vi "Test CIF pcap PubSub.vi"() -> ()   [LabVIEW 2021]
uses:
  typedef/CIF Pcap Publisher Configuration.ctl
  typedef/CIF Pcap Subscriber Configuration.ctl
  typedef/CIF Channel Header Publisher.ctl
  typedef/CIF Channel Header.ctl
  typedef/Publisher Info.ctl
  typedef/CIF Pcap Publish Advanced.ctl
  typedef/CIF Pcap Publisher Stats.ctl
  typedef/CIF Pcap Subscriber Stats.ctl
  SubVIs/Get Path.vi
  SubVIs/Convert Error.vi
  SubVIs/Add Error.vi
  Refnum/CIF Publisher to Refnum.vi
  <vilib>/CIF Foundation/CIF Utilities/File/File/File Not Found Error Update.vi
  Refnum/CIF Subscriber to Refnum.vi
  SubVIs/Check data length for publish.vi
  Refnum/CIF Publisher from Refnum.vi
  Refnum/CIF Subscriber from Refnum.vi
  <vilib>/Utility/error.llb/Trim Whitespace.vi
  SubVIs/Add Error Core.vi
  SubVIs/Convert Error Core.vi
  <vilib>/CIF Foundation/CIF Utilities/File/SubVIs/File Not Found Error Core.vi
  Iceoryx.lvlib
panel:
  out "status":string
  out "pass":bool
  out "error out":errorcluster
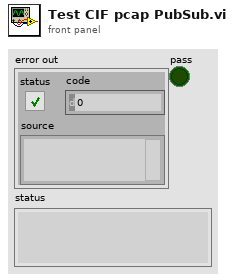
[diagram p1: front panel]
types:
  T1 = typedef "Iceoryx.lvlib/CIF Channel Header.ctl" = cluster{"Length":u64, "T0":i64, "T_Out":i64, "T_Tx":i64, "Ctr":u64, "ClockID":u8}
  T2 = typedef "Iceoryx.lvlib/CIF Channel Header Publisher.ctl" = cluster{"T0":i64, "T_Out":i64, "T_Tx":i64, "ClockID":u8}
  T3 = typedef "Iceoryx.lvlib/CIF Pcap Subscriber Configuration.ctl" = cluster{"Name":string, "Topic":string, "Link Type":u32, "Backpressure":bool}
  T4 = typedef "Iceoryx.lvlib/CIF Pcap Publisher Configuration.ctl" = cluster{"Name":string, "Topic":string, "Link Type":u32, "Descriptor":string, "Max Bytes":u32, "Best Effort Subscribers":u32, "Backpressure Subscribers":u32, "Best Effort Queue Depth":u32, "Backpressure Queue Depth":u32}
  T5 = typedef "Iceoryx.lvlib/Publisher Info.ctl" = cluster{"Type":string, "Element Size":u32, "Max Elements in Array":u32, "Backpressure Queue Depth":u32, "Best Effort Queue Depth":u32}
  T6 = typedef "Iceoryx.lvlib/CIF Pcap Publish Advanced.ctl" = cluster{"Offset":u32, "Length":i32}
  T7 = typedef "Iceoryx.lvlib/CIF Pcap Publisher Stats.ctl" = cluster{"Writes":u64, "TX Timeouts":u64}
  T8 = typedef "Iceoryx.lvlib/CIF Pcap Subscriber Stats.ctl" = cluster{"Reads":u64, "RX Timeouts":u64, "Dropped":u64}
  T9 = typedef "Iceoryx.lvlib/CIF Publisher Refnum.ctl" = cluster{"refnum":u64, "CIF Pub":enum8{"cifpub"}}
  T10 = typedef "Iceoryx.lvlib/CIF Subscriber Refnum.ctl" = cluster{"refnum":u64, "CIF Sub":enum8{"cifsub"}}
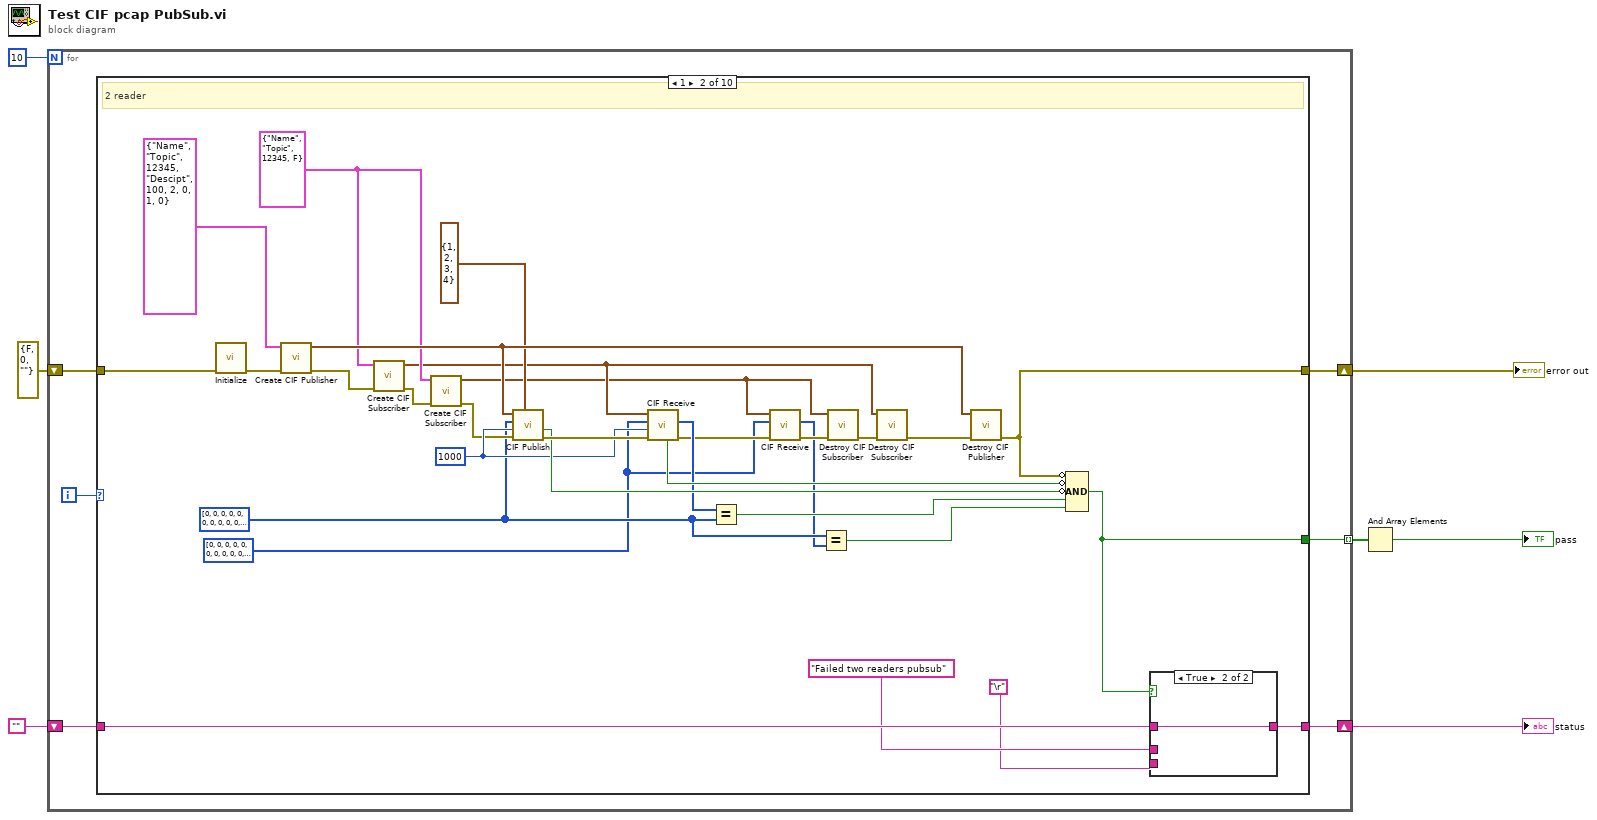
[diagram p0: block diagram]
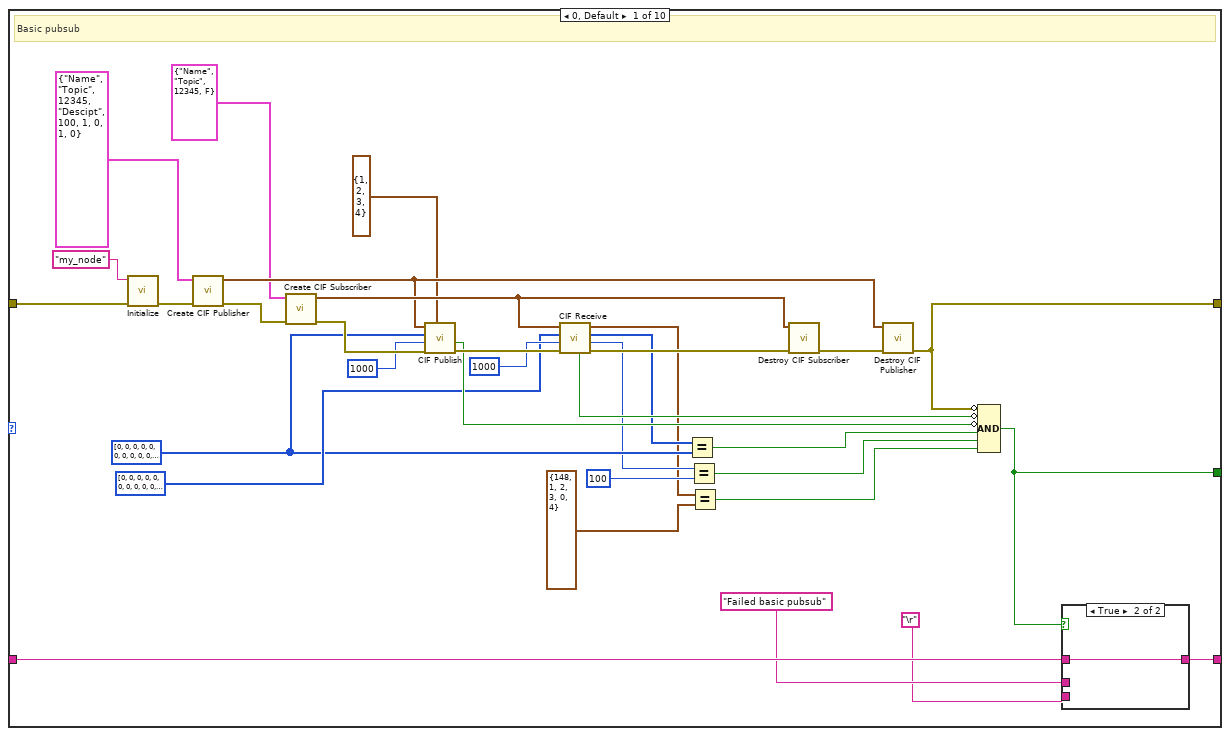
[diagram p2: hidden frame]
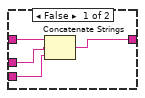
[diagram p3: hidden frame]
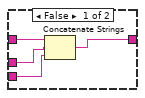
[diagram p4: hidden frame]
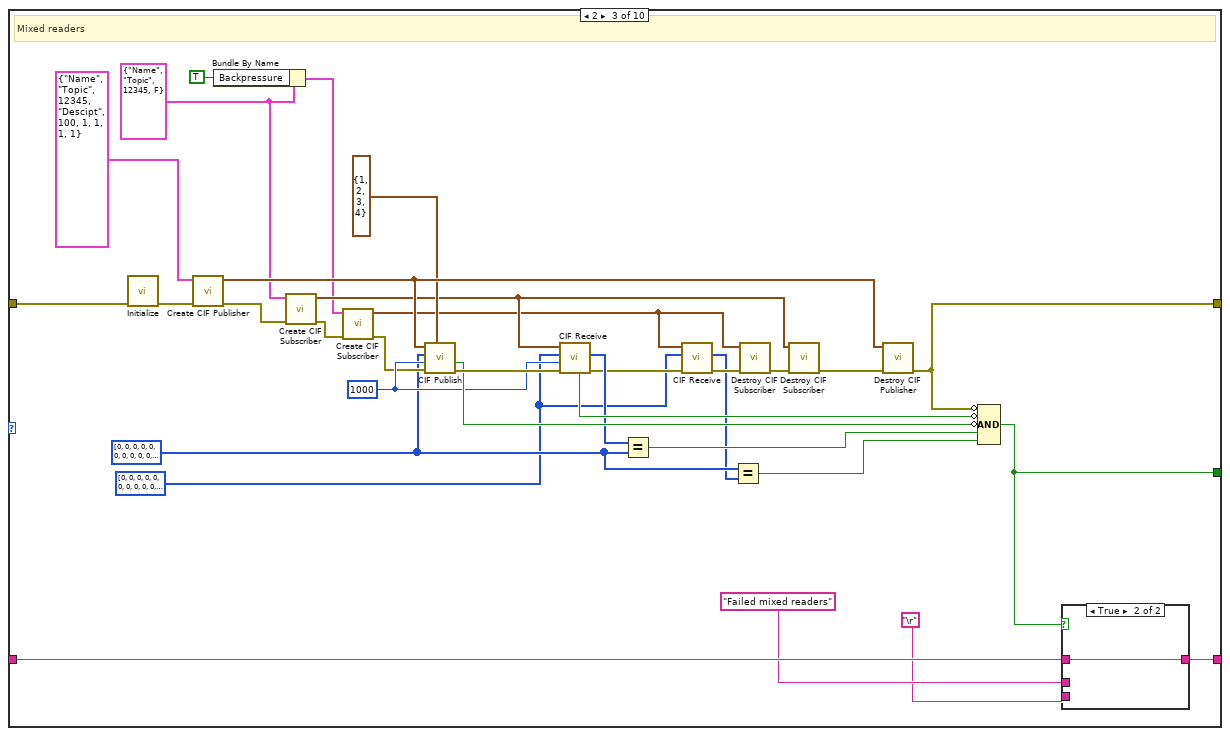
[diagram p5: hidden frame]
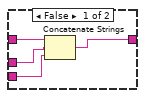
[diagram p6: hidden frame]
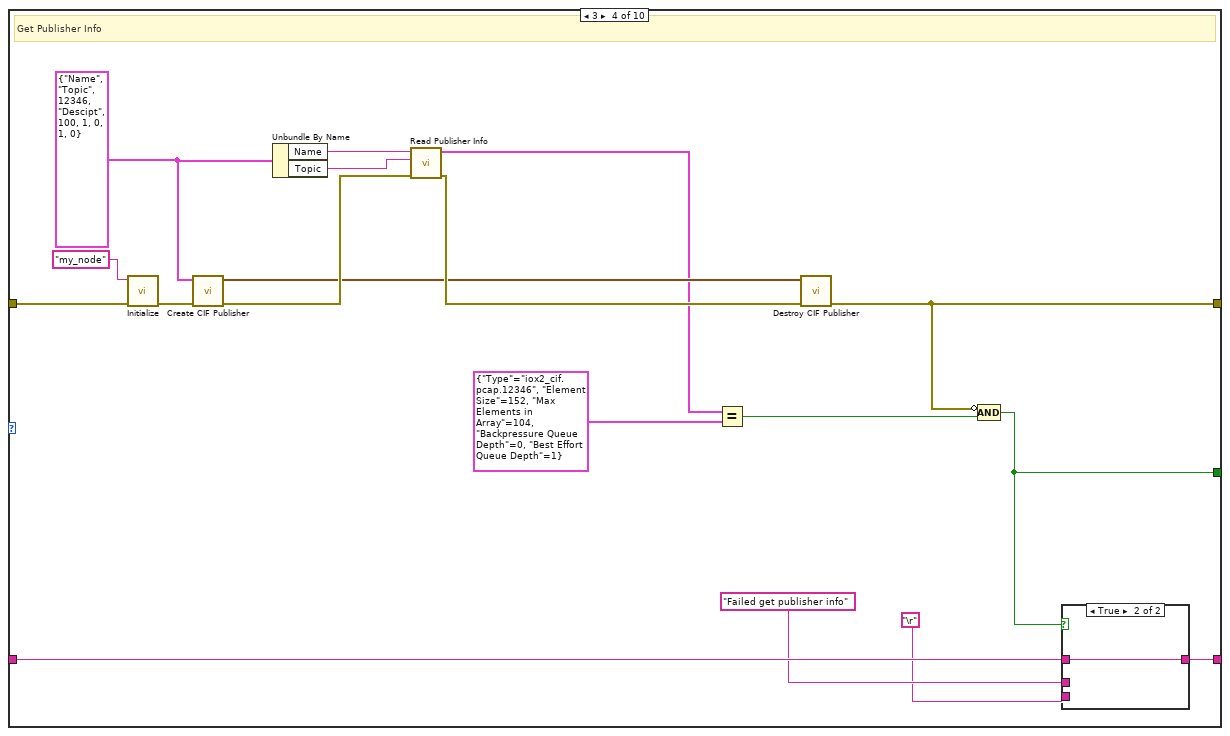
[diagram p7: hidden frame]
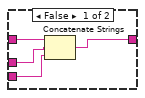
[diagram p8: hidden frame]
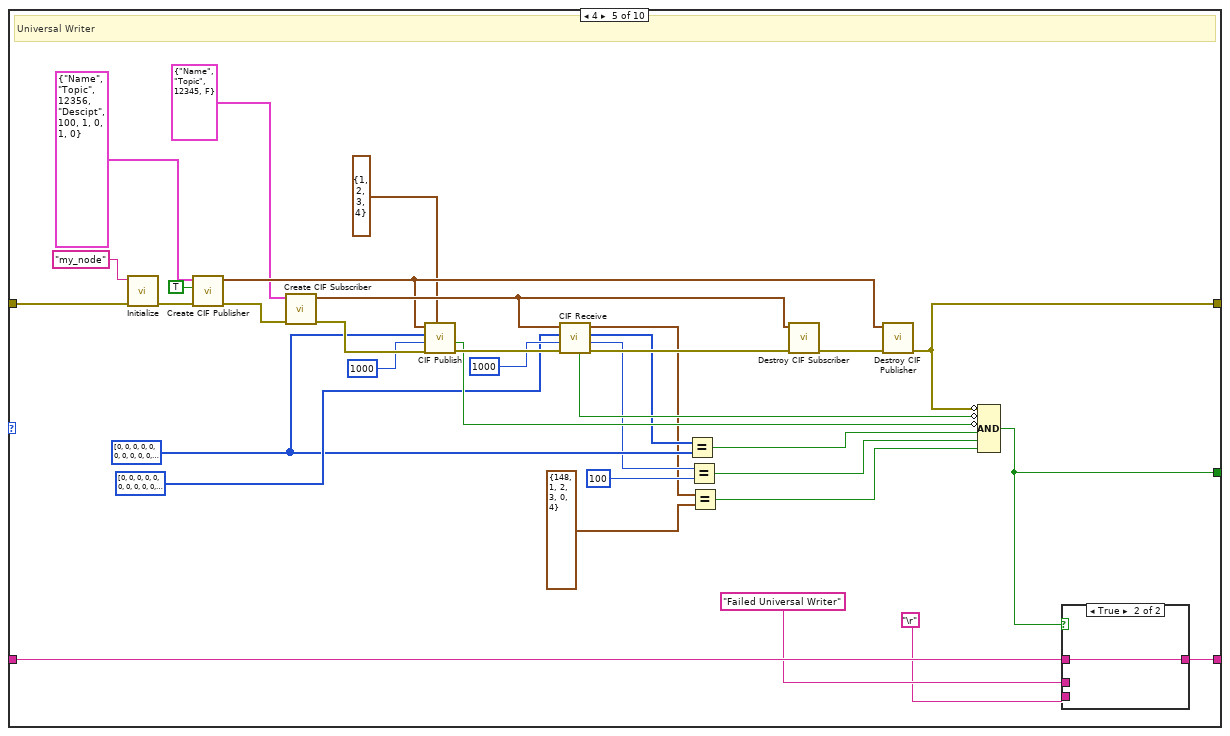
[diagram p9: hidden frame]
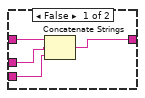
[diagram p10: hidden frame]
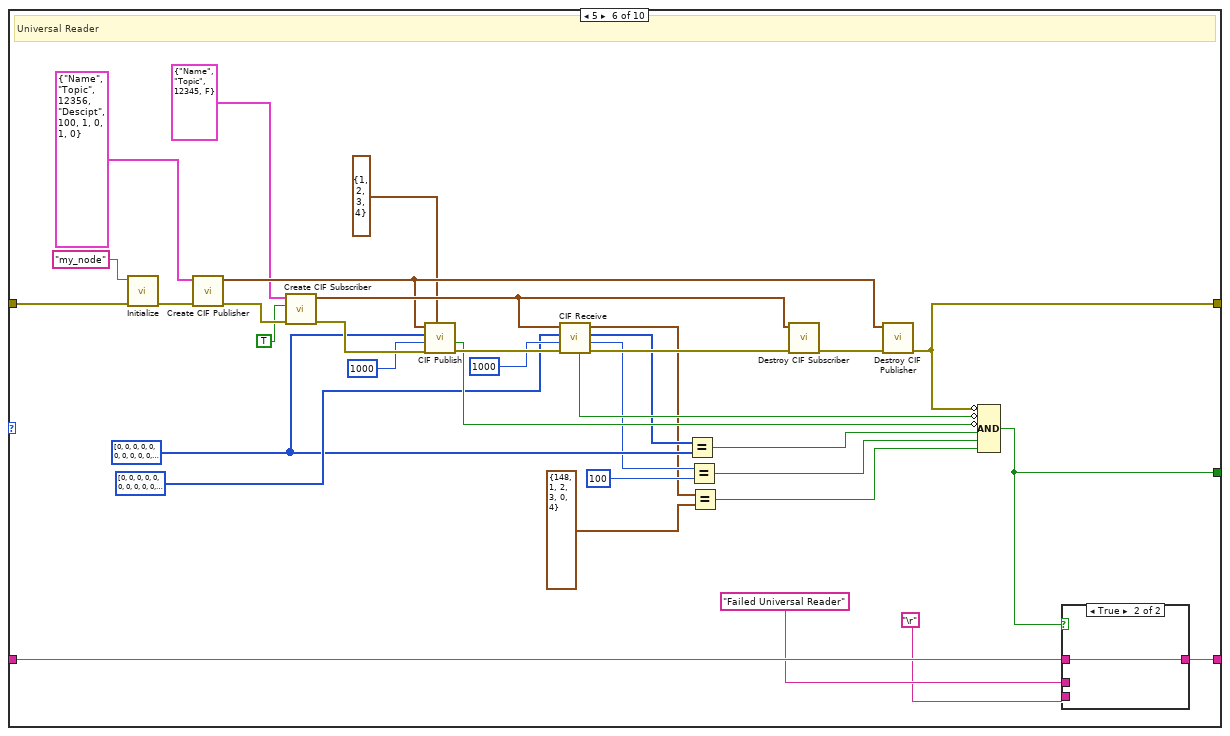
[diagram p11: hidden frame]
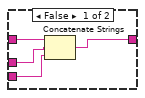
[diagram p12: hidden frame]
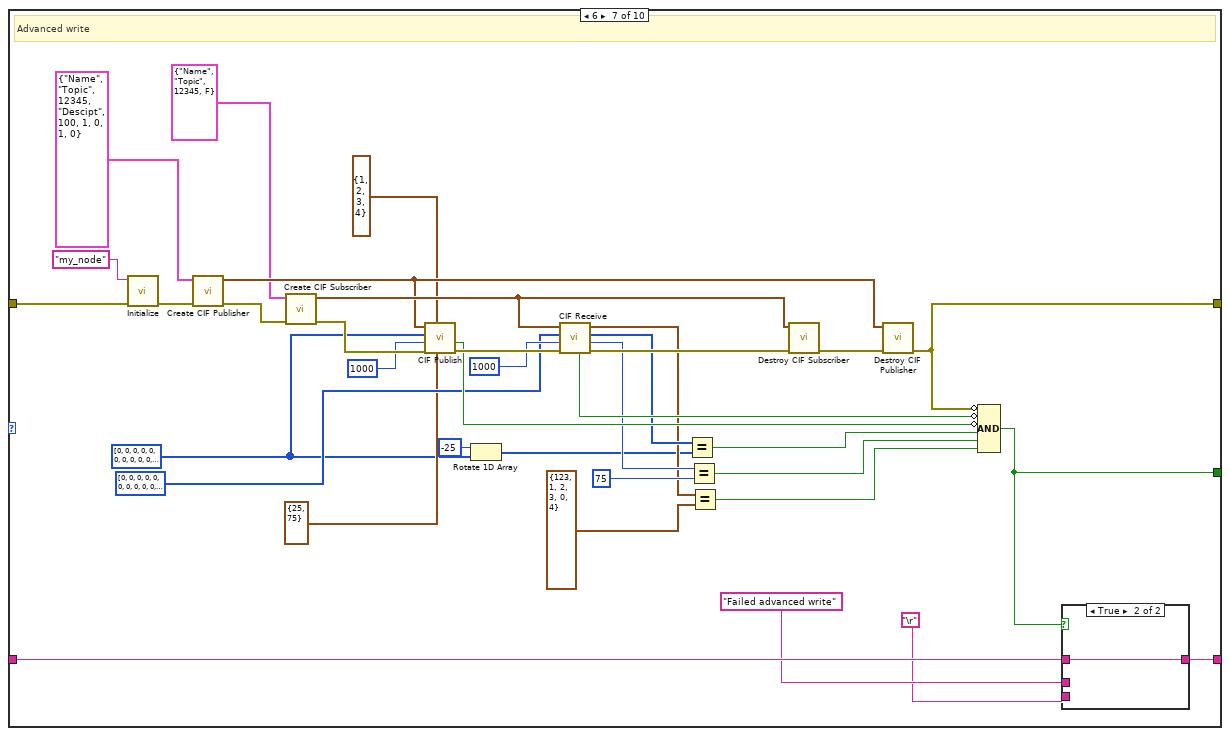
[diagram p13: hidden frame]
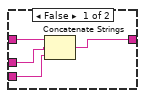
[diagram p14: hidden frame]
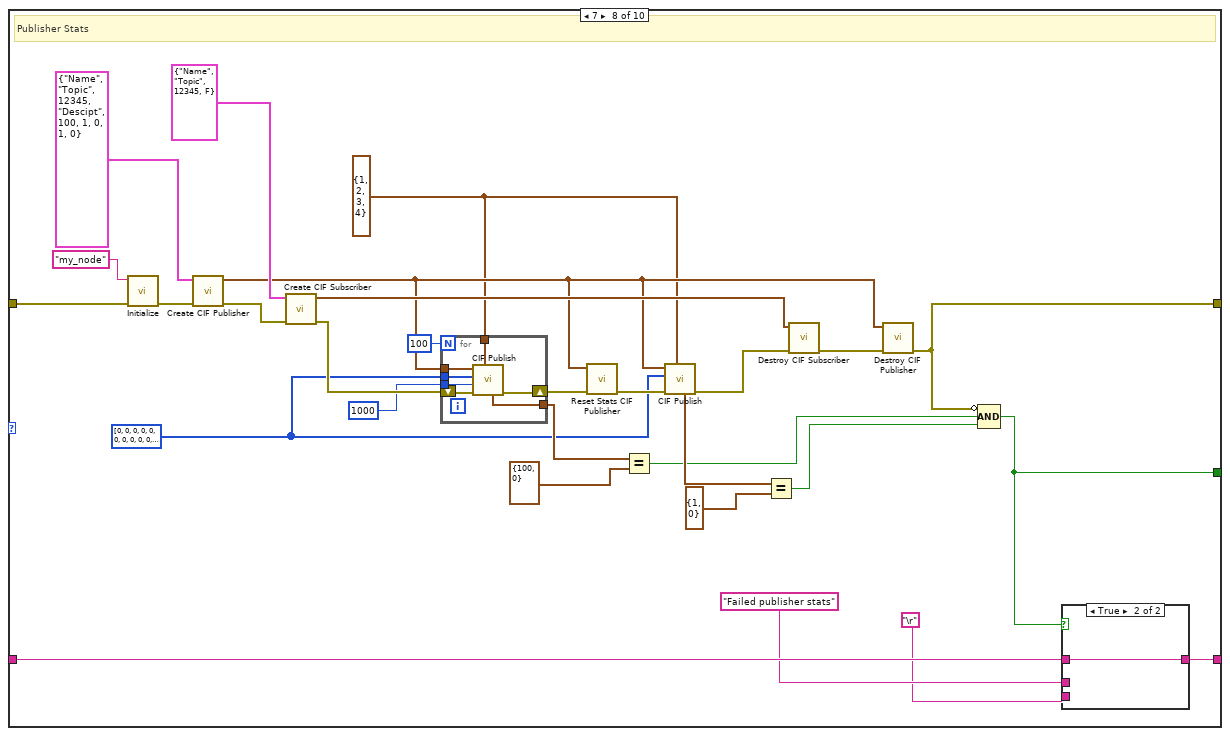
[diagram p15: hidden frame]
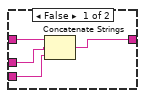
[diagram p16: hidden frame]
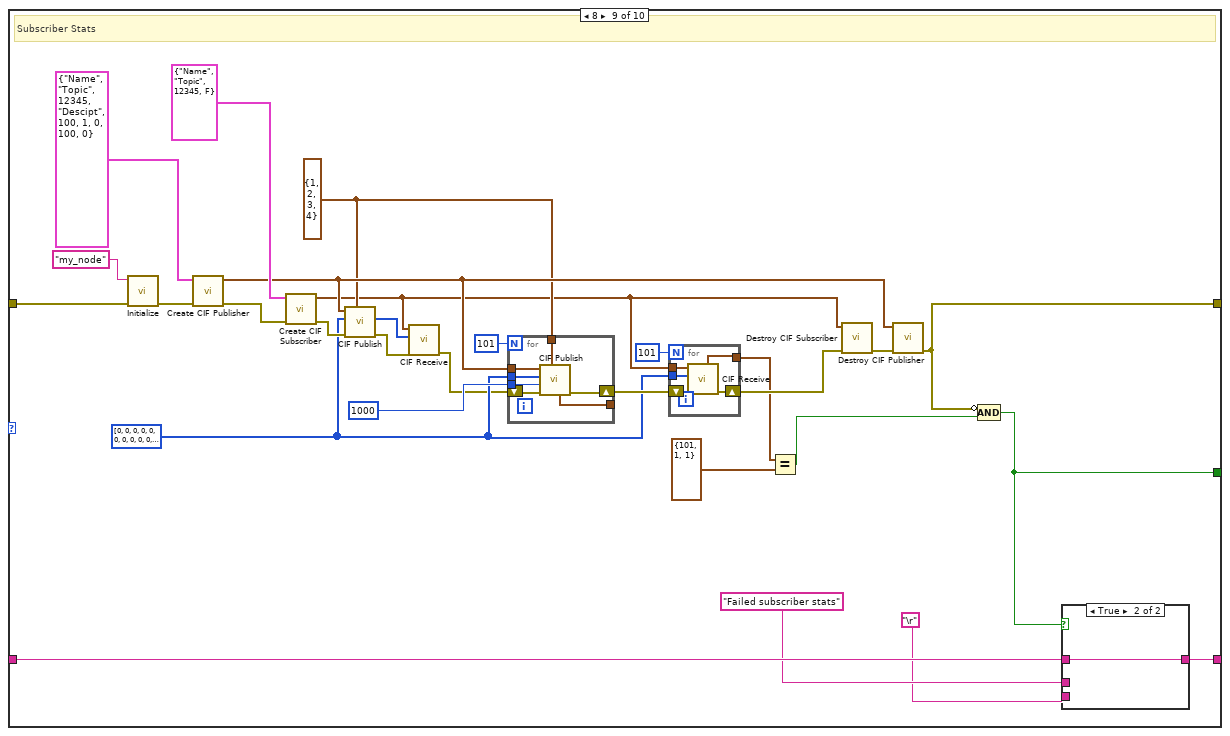
[diagram p17: hidden frame]
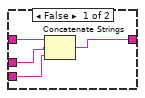
[diagram p18: hidden frame]
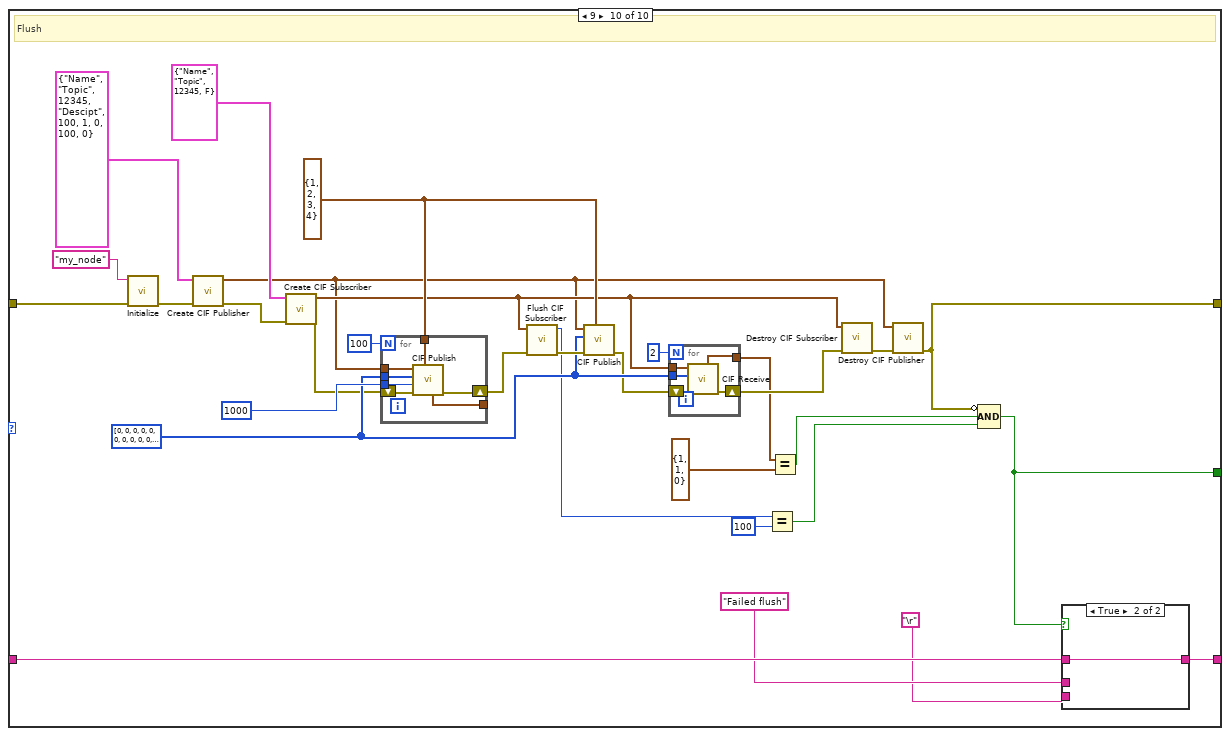
[diagram p19: hidden frame]
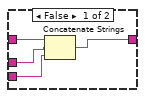
[diagram p20: hidden frame]
diagram:
  n1 = for {
    N: 10 -> [_]
    tunnel: [w13] -> w7 mode=indexing
    shift-right: [w10] -> w3
    shift-left: "" -> [w11]
    shift-right: [w9] -> w1
    shift-left: errorcluster {"status"=FALSE, "code"=0, "source"=""} ("error out") -> [w8]
    i -> [w12]
    n2 = case shown="1" w12 {
      tunnel: [w42 w78 w116 w139 w178 w217 w258 w292 w333 w381] -> w13
      tunnel: w11 -> [w46 w82 w120 w143 w182 w221 w262 w296 w337 w385]
      tunnel: [w45 w81 w119 w142 w181 w220 w261 w295 w336 w384] -> w10
      tunnel: [w31 w71 w109 w129 w167 w206 w247 w284 w327 w375] -> w9
      tunnel: w8 -> [w41 w77 w115 w138 w177 w216 w257 w291 w332 w380]
      frame 0, Default {
        w20 = u8[] [0, 0, 0, 0, 0, 0, 0, 0, 0, 0, 0, 0, 0, 0, 0, 0, 0, 0, 0, 0, 0, 0, 0, 0, 0, 0, 0, 0, 0, 0, 0, 0, 0, 0, 0, 0, 0, 0, 0, 0, 0, 0, 0, 0, 0, 0, 0, 0, 0, 0, 0, 0, 0, 0, 0, 0, 0, 0, 0, 0, 0, 0, 0, 0, 0, 0, 0, 0, 0, 0, 0, 0, 0, 0, 0, 0, 0, 0, 0, 0, 0, 0, 0, 0, 0, 0, 0, 0, 0, 0, 0, 0, 0, 0, 0, 0, 0, 0, 0, 1] ("Data In")
        # "Basic pubsub"
        n3 = call "Initialize.vi"("error in (no error)"=w41, "Node name"="my_node") -> ("error out"=w39:errorcluster)  [unwired: 9 in]
        n4 = call "Create CIF Publisher.vi"("error in (no error)"=w39, "CIF Pcap Publisher Configuration"=T4 {"Name"="Name", "Topic"="Topic", "Link Type"=12345, "Descriptor"="Descipt", "Max Bytes"=100, "Best Effort Subscribers"=1, "Backpressure Subscribers"=0, "Best Effort Queue Depth"=1, "Backpressure Queue Depth"=0}) -> ("error out"=w38:errorcluster, "CIF Publisher Refnum"=w32:T9)  [unwired: 8 in]
        n5 = call "Create CIF Subscriber.vi"("error in (no error)"=w38, "CIF Pcap Subscriber Configuration"=T3 {"Name"="Name", "Topic"="Topic", "Link Type"=12345, "Backpressure"=FALSE}) -> ("error out"=w37:errorcluster, "CIF Subscriber Refnum"=w34:T10)  [unwired: 8 in]
        n6 = call "CIF Publish.vi"("CIF Channel Header Publisher"=T2 {"T0"=1, "T_Out"=2, "T_Tx"=3, "ClockID"=4}, "error in (no error)"=w37, "Timeout ms"=u32 1000 ("Timoeut ms"), "Data In"=w20, "Publisher Reference"=w32) -> ("error out"=w36:errorcluster, "Timeout"=w27:bool)  [unwired: 3 in, 2 out]
        n7 = call "CIF Receive.vi"("error in (no error)"=w36, "Timoeut ms"=u32 1000, "Data In"=u8[] [0, 0, 0, 0, 0, 0, 0, 0, 0, 0, 0, 0, 0, 0, 0, 0, 0, 0, 0, 0, 0, 0, 0, 0, 0, 0, 0, 0, 0, 0, 0, 0, 0, 0, 0, 0, 0, 0, 0, 0, 0, 0, 0, 0, 0, 0, 0, 0, 0, 0, 0, 0, 0, 0, 0, 0, 0, 0, 0, 0, 0, 0, 0, 0, 0, 0, 0, 0, 0, 0, 0, 0, 0, 0, 0, 0, 0, 0, 0, 0, 0, 0, 0, 0, 0, 0, 0, 0, 0, 0, 0, 0, 0, 0, 0, 0, 0, 0, 0, 0], "Subscriber Reference"=w34) -> ("error out"=w35:errorcluster, "Array Length"=w19:u32, "Data Out"=w21:u8[], "CIF Channel Header"=w16:T1, "Timeout"=w26:bool)  [unwired: 2 in, 1 out]
        n8 = Equal?(x=w21, y=w20) -> (x = y?=w28:bool)
        n9 = Equal?(x=w19, y=u32 100) -> (x = y?=w17:bool)
        n10 = Equal?(x=w16, y=T1 {"Length"=148, "T0"=1, "T_Out"=2, "T_Tx"=3, "Ctr"=0, "ClockID"=4} ("CIF Channel Header")) -> (x = y?=w15:bool)
        n11 = call "Destroy CIF Subscriber.vi"("error in (no error)"=w35, "Subscriber Reference"=w34) -> ("error out"=w33:errorcluster)  [unwired: 9 in]
        n12 = call "Destroy CIF Publisher.vi"("error in (no error)"=w33, "Publisher Reference"=w32) -> ("error out"=w31:errorcluster)  [unwired: 9 in]
        n13 = Compound Arithmetic op=AND(invert w31, invert w26, invert w27, w28, w17, w15) -> (w42:bool)
        n14 = case shown="True" w42 {
          tunnel: w46 -> [w50 w51]
          tunnel: [w47 w51] -> w45
          tunnel: "Failed basic pubsub" -> [w49 _]
          tunnel: "\r" -> [w48 _]
          frame False {
            n15 = Concatenate Strings(w50, w49, w48) -> (w47:string)
          }
          frame True {
          }
        }
      }
      frame 1 {
        w52 = u8[] [0, 0, 0, 0, 0, 0, 0, 0, 0, 0, 0, 0, 0, 0, 0, 0, 0, 0, 0, 0, 0, 0, 0, 0, 0, 0, 0, 0, 0, 0, 0, 0, 0, 0, 0, 0, 0, 0, 0, 0, 0, 0, 0, 0, 0, 0, 0, 0, 0, 0, 0, 0, 0, 0, 0, 0, 0, 0, 0, 0, 0, 0, 0, 0, 0, 0, 0, 0, 0, 0, 0, 0, 0, 0, 0, 0, 0, 0, 0, 0, 0, 0, 0, 0, 0, 0, 0, 0, 0, 0, 0, 0, 0, 0, 0, 0, 0, 0, 0, 0] ("Data In")
        w55 = u8[] [0, 0, 0, 0, 0, 0, 0, 0, 0, 0, 0, 0, 0, 0, 0, 0, 0, 0, 0, 0, 0, 0, 0, 0, 0, 0, 0, 0, 0, 0, 0, 0, 0, 0, 0, 0, 0, 0, 0, 0, 0, 0, 0, 0, 0, 0, 0, 0, 0, 0, 0, 0, 0, 0, 0, 0, 0, 0, 0, 0, 0, 0, 0, 0, 0, 0, 0, 0, 0, 0, 0, 0, 0, 0, 0, 0, 0, 0, 0, 0, 0, 0, 0, 0, 0, 0, 0, 0, 0, 0, 0, 0, 0, 0, 0, 0, 0, 0, 0, 1] ("Data In")
        w60 = T3 {"Name"="Name", "Topic"="Topic", "Link Type"=12345, "Backpressure"=FALSE} ("CIF Pcap Subscriber Configuration")
        w63 = u32 1000 ("Timoeut ms")
        # "2 reader"
        n16 = call "Initialize.vi"("error in (no error)"=w77) -> ("error out"=w76:errorcluster)  [unwired: 10 in]
        n17 = call "Create CIF Publisher.vi"("error in (no error)"=w76, "CIF Pcap Publisher Configuration"=T4 {"Name"="Name", "Topic"="Topic", "Link Type"=12345, "Descriptor"="Descipt", "Max Bytes"=100, "Best Effort Subscribers"=2, "Backpressure Subscribers"=0, "Best Effort Queue Depth"=1, "Backpressure Queue Depth"=0}) -> ("error out"=w75:errorcluster, "CIF Publisher Refnum"=w72:T9)  [unwired: 8 in]
        n18 = call "Create CIF Subscriber.vi"("error in (no error)"=w75, "CIF Pcap Subscriber Configuration"=w60) -> ("error out"=w62:errorcluster, "CIF Subscriber Refnum"=w56:T10)  [unwired: 8 in]
        n19 = call "Create CIF Subscriber.vi"("error in (no error)"=w62, "CIF Pcap Subscriber Configuration"=w60) -> ("error out"=w61:errorcluster, "CIF Subscriber Refnum"=w53:T10)  [unwired: 8 in]
        n20 = call "CIF Publish.vi"("CIF Channel Header Publisher"=T2 {"T0"=1, "T_Out"=2, "T_Tx"=3, "ClockID"=4}, "error in (no error)"=w61, "Timeout ms"=w63, "Data In"=w55, "Publisher Reference"=w72) -> ("error out"=w74:errorcluster, "Timeout"=w69:bool)  [unwired: 3 in, 2 out]
        n21 = call "CIF Receive.vi"("error in (no error)"=w74, "Timoeut ms"=w63, "Data In"=w52, "Subscriber Reference"=w56) -> ("error out"=w59:errorcluster, "Data Out"=w65:u8[], "Timeout"=w68:bool)  [unwired: 2 in, 3 out]
        n22 = Equal?(x=w65, y=w55) -> (x = y?=w70:bool)
        n23 = call "CIF Receive.vi"("error in (no error)"=w59, "Data In"=w52, "Subscriber Reference"=w53) -> ("error out"=w58:errorcluster, "Data Out"=w54:u8[])  [unwired: 3 in, 4 out]
        n24 = Equal?(x=w55, y=w54) -> (x = y?=w64:bool)
        n25 = call "Destroy CIF Subscriber.vi"("error in (no error)"=w58, "Subscriber Reference"=w53) -> ("error out"=w57:errorcluster)  [unwired: 9 in]
        n26 = call "Destroy CIF Subscriber.vi"("error in (no error)"=w57, "Subscriber Reference"=w56) -> ("error out"=w73:errorcluster)  [unwired: 9 in]
        n27 = call "Destroy CIF Publisher.vi"("error in (no error)"=w73, "Publisher Reference"=w72) -> ("error out"=w71:errorcluster)  [unwired: 9 in]
        n28 = Compound Arithmetic op=AND(invert w71, invert w68, invert w69, w70, w64) -> (w78:bool)
        n29 = case shown="True" w78 {
          tunnel: w82 -> [w86 w87]
          tunnel: [w83 w87] -> w81
          tunnel: "Failed two readers pubsub" -> [w85 _]
          tunnel: "\r" -> [w84 _]
          frame False {
            n30 = Concatenate Strings(w86, w85, w84) -> (w83:string)
          }
          frame True {
          }
        }
      }
      frame 2 {
        w91 = u8[] [0, 0, 0, 0, 0, 0, 0, 0, 0, 0, 0, 0, 0, 0, 0, 0, 0, 0, 0, 0, 0, 0, 0, 0, 0, 0, 0, 0, 0, 0, 0, 0, 0, 0, 0, 0, 0, 0, 0, 0, 0, 0, 0, 0, 0, 0, 0, 0, 0, 0, 0, 0, 0, 0, 0, 0, 0, 0, 0, 0, 0, 0, 0, 0, 0, 0, 0, 0, 0, 0, 0, 0, 0, 0, 0, 0, 0, 0, 0, 0, 0, 0, 0, 0, 0, 0, 0, 0, 0, 0, 0, 0, 0, 0, 0, 0, 0, 0, 0, 0] ("Data In")
        w94 = u8[] [0, 0, 0, 0, 0, 0, 0, 0, 0, 0, 0, 0, 0, 0, 0, 0, 0, 0, 0, 0, 0, 0, 0, 0, 0, 0, 0, 0, 0, 0, 0, 0, 0, 0, 0, 0, 0, 0, 0, 0, 0, 0, 0, 0, 0, 0, 0, 0, 0, 0, 0, 0, 0, 0, 0, 0, 0, 0, 0, 0, 0, 0, 0, 0, 0, 0, 0, 0, 0, 0, 0, 0, 0, 0, 0, 0, 0, 0, 0, 0, 0, 0, 0, 0, 0, 0, 0, 0, 0, 0, 0, 0, 0, 0, 0, 0, 0, 0, 0, 1] ("Data In")
        w89 = T3 {"Name"="Name", "Topic"="Topic", "Link Type"=12345, "Backpressure"=FALSE} ("CIF Pcap Subscriber Configuration")
        w101 = u32 1000 ("Timoeut ms")
        # "Mixed readers"
        n31 = call "Initialize.vi"("error in (no error)"=w115) -> ("error out"=w114:errorcluster)  [unwired: 10 in]
        n32 = call "Create CIF Publisher.vi"("error in (no error)"=w114, "CIF Pcap Publisher Configuration"=T4 {"Name"="Name", "Topic"="Topic", "Link Type"=12345, "Descriptor"="Descipt", "Max Bytes"=100, "Best Effort Subscribers"=1, "Backpressure Subscribers"=1, "Best Effort Queue Depth"=1, "Backpressure Queue Depth"=1}) -> ("error out"=w113:errorcluster, "CIF Publisher Refnum"=w110:T9)  [unwired: 8 in]
        n33 = Bundle By Name(cluster=w89, "Backpressure"=TRUE) -> (w88:T3)
        n34 = call "Create CIF Subscriber.vi"("error in (no error)"=w113, "CIF Pcap Subscriber Configuration"=w89) -> ("error out"=w100:errorcluster, "CIF Subscriber Refnum"=w95:T10)  [unwired: 8 in]
        n35 = call "Create CIF Subscriber.vi"("error in (no error)"=w100, "CIF Pcap Subscriber Configuration"=w88) -> ("error out"=w99:errorcluster, "CIF Subscriber Refnum"=w92:T10)  [unwired: 8 in]
        n36 = call "CIF Publish.vi"("CIF Channel Header Publisher"=T2 {"T0"=1, "T_Out"=2, "T_Tx"=3, "ClockID"=4}, "error in (no error)"=w99, "Timeout ms"=w101, "Data In"=w94, "Publisher Reference"=w110) -> ("error out"=w112:errorcluster, "Timeout"=w107:bool)  [unwired: 3 in, 2 out]
        n37 = call "CIF Receive.vi"("error in (no error)"=w112, "Timoeut ms"=w101, "Data In"=w91, "Subscriber Reference"=w95) -> ("error out"=w98:errorcluster, "Data Out"=w103:u8[], "Timeout"=w106:bool)  [unwired: 2 in, 3 out]
        n38 = Equal?(x=w103, y=w94) -> (x = y?=w108:bool)
        n39 = call "CIF Receive.vi"("error in (no error)"=w98, "Data In"=w91, "Subscriber Reference"=w92) -> ("error out"=w97:errorcluster, "Data Out"=w93:u8[])  [unwired: 3 in, 4 out]
        n40 = Equal?(x=w94, y=w93) -> (x = y?=w102:bool)
        n41 = call "Destroy CIF Subscriber.vi"("error in (no error)"=w97, "Subscriber Reference"=w92) -> ("error out"=w96:errorcluster)  [unwired: 9 in]
        n42 = call "Destroy CIF Subscriber.vi"("error in (no error)"=w96, "Subscriber Reference"=w95) -> ("error out"=w111:errorcluster)  [unwired: 9 in]
        n43 = call "Destroy CIF Publisher.vi"("error in (no error)"=w111, "Publisher Reference"=w110) -> ("error out"=w109:errorcluster)  [unwired: 9 in]
        n44 = Compound Arithmetic op=AND(invert w109, invert w106, invert w107, w108, w102) -> (w116:bool)
        n45 = case shown="True" w116 {
          tunnel: w120 -> [w124 w125]
          tunnel: [w121 w125] -> w119
          tunnel: "Failed mixed readers" -> [w123 _]
          tunnel: "\r" -> [w122 _]
          frame False {
            n46 = Concatenate Strings(w124, w123, w122) -> (w121:string)
          }
          frame True {
          }
        }
      }
      frame 3 {
        w132 = T4 {"Name"="Name", "Topic"="Topic", "Link Type"=12346, "Descriptor"="Descipt", "Max Bytes"=100, "Best Effort Subscribers"=1, "Backpressure Subscribers"=0, "Best Effort Queue Depth"=1, "Backpressure Queue Depth"=0} ("CIF Pcap Publisher Configuration")
        # "Get Publisher Info"
        n47 = call "Initialize.vi"("error in (no error)"=w138, "Node name"="my_node") -> ("error out"=w136:errorcluster)  [unwired: 9 in]
        n48 = call "Create CIF Publisher.vi"("error in (no error)"=w136, "CIF Pcap Publisher Configuration"=w132) -> ("error out"=w131:errorcluster, "CIF Publisher Refnum"=w128:T9)  [unwired: 8 in]
        n49 = Unbundle By Name(w132) -> ("Name"=w134:string, "Topic"=w133:string)
        n50 = call "Read Publisher Info.vi"("error in (no error)"=w131, "Topic"=w133, "Name"=w134) -> ("error out"=w130:errorcluster, "Publisher Info"=w127:T5)  [unwired: 7 in]
        n51 = Equal?(x=w127, y=T5 {"Type"="iox2_cif.pcap.12346", "Element Size"=152, "Max Elements in Array"=104, "Backpressure Queue Depth"=0, "Best Effort Queue Depth"=1} ("Publisher Info")) -> (x = y?=w135:bool)
        n52 = call "Destroy CIF Publisher.vi"("error in (no error)"=w130, "Publisher Reference"=w128) -> ("error out"=w129:errorcluster)  [unwired: 9 in]
        n53 = Compound Arithmetic op=AND(invert w129, w135) -> (w139:bool)
        n54 = case shown="True" w139 {
          tunnel: w143 -> [w147 w148]
          tunnel: [w144 w148] -> w142
          tunnel: "Failed get publisher info" -> [w146 _]
          tunnel: "\r" -> [w145 _]
          frame False {
            n55 = Concatenate Strings(w147, w146, w145) -> (w144:string)
          }
          frame True {
          }
        }
      }
      frame 4 {
        w156 = u8[] [0, 0, 0, 0, 0, 0, 0, 0, 0, 0, 0, 0, 0, 0, 0, 0, 0, 0, 0, 0, 0, 0, 0, 0, 0, 0, 0, 0, 0, 0, 0, 0, 0, 0, 0, 0, 0, 0, 0, 0, 0, 0, 0, 0, 0, 0, 0, 0, 0, 0, 0, 0, 0, 0, 0, 0, 0, 0, 0, 0, 0, 0, 0, 0, 0, 0, 0, 0, 0, 0, 0, 0, 0, 0, 0, 0, 0, 0, 0, 0, 0, 0, 0, 0, 0, 0, 0, 0, 0, 0, 0, 0, 0, 0, 0, 0, 0, 0, 0, 1] ("Data In")
        # "Universal Writer"
        n56 = call "Initialize.vi"("error in (no error)"=w177, "Node name"="my_node") -> ("error out"=w175:errorcluster)  [unwired: 9 in]
        n57 = call "Create CIF Publisher.vi"("error in (no error)"=w175, "Universal"=TRUE, "CIF Pcap Publisher Configuration"=T4 {"Name"="Name", "Topic"="Topic", "Link Type"=12356, "Descriptor"="Descipt", "Max Bytes"=100, "Best Effort Subscribers"=1, "Backpressure Subscribers"=0, "Best Effort Queue Depth"=1, "Backpressure Queue Depth"=0}) -> ("error out"=w174:errorcluster, "CIF Publisher Refnum"=w168:T9)  [unwired: 7 in]
        n58 = call "Create CIF Subscriber.vi"("error in (no error)"=w174, "CIF Pcap Subscriber Configuration"=T3 {"Name"="Name", "Topic"="Topic", "Link Type"=12345, "Backpressure"=FALSE}) -> ("error out"=w173:errorcluster, "CIF Subscriber Refnum"=w170:T10)  [unwired: 8 in]
        n59 = call "CIF Publish.vi"("CIF Channel Header Publisher"=T2 {"T0"=1, "T_Out"=2, "T_Tx"=3, "ClockID"=4}, "error in (no error)"=w173, "Timeout ms"=u32 1000 ("Timoeut ms"), "Data In"=w156, "Publisher Reference"=w168) -> ("error out"=w172:errorcluster, "Timeout"=w163:bool)  [unwired: 3 in, 2 out]
        n60 = call "CIF Receive.vi"("error in (no error)"=w172, "Timoeut ms"=u32 1000, "Data In"=u8[] [0, 0, 0, 0, 0, 0, 0, 0, 0, 0, 0, 0, 0, 0, 0, 0, 0, 0, 0, 0, 0, 0, 0, 0, 0, 0, 0, 0, 0, 0, 0, 0, 0, 0, 0, 0, 0, 0, 0, 0, 0, 0, 0, 0, 0, 0, 0, 0, 0, 0, 0, 0, 0, 0, 0, 0, 0, 0, 0, 0, 0, 0, 0, 0, 0, 0, 0, 0, 0, 0, 0, 0, 0, 0, 0, 0, 0, 0, 0, 0, 0, 0, 0, 0, 0, 0, 0, 0, 0, 0, 0, 0, 0, 0, 0, 0, 0, 0, 0, 0], "Subscriber Reference"=w170) -> ("error out"=w171:errorcluster, "Array Length"=w155:u32, "Data Out"=w157:u8[], "CIF Channel Header"=w152:T1, "Timeout"=w162:bool)  [unwired: 2 in, 1 out]
        n61 = Equal?(x=w157, y=w156) -> (x = y?=w164:bool)
        n62 = Equal?(x=w155, y=u32 100) -> (x = y?=w153:bool)
        n63 = Equal?(x=w152, y=T1 {"Length"=148, "T0"=1, "T_Out"=2, "T_Tx"=3, "Ctr"=0, "ClockID"=4} ("CIF Channel Header")) -> (x = y?=w151:bool)
        n64 = call "Destroy CIF Subscriber.vi"("error in (no error)"=w171, "Subscriber Reference"=w170) -> ("error out"=w169:errorcluster)  [unwired: 9 in]
        n65 = call "Destroy CIF Publisher.vi"("error in (no error)"=w169, "Publisher Reference"=w168) -> ("error out"=w167:errorcluster)  [unwired: 9 in]
        n66 = Compound Arithmetic op=AND(invert w167, invert w162, invert w163, w164, w153, w151) -> (w178:bool)
        n67 = case shown="True" w178 {
          tunnel: w182 -> [w186 w187]
          tunnel: [w183 w187] -> w181
          tunnel: "Failed Universal Writer" -> [w185 _]
          tunnel: "\r" -> [w184 _]
          frame False {
            n68 = Concatenate Strings(w186, w185, w184) -> (w183:string)
          }
          frame True {
          }
        }
      }
      frame 5 {
        w195 = u8[] [0, 0, 0, 0, 0, 0, 0, 0, 0, 0, 0, 0, 0, 0, 0, 0, 0, 0, 0, 0, 0, 0, 0, 0, 0, 0, 0, 0, 0, 0, 0, 0, 0, 0, 0, 0, 0, 0, 0, 0, 0, 0, 0, 0, 0, 0, 0, 0, 0, 0, 0, 0, 0, 0, 0, 0, 0, 0, 0, 0, 0, 0, 0, 0, 0, 0, 0, 0, 0, 0, 0, 0, 0, 0, 0, 0, 0, 0, 0, 0, 0, 0, 0, 0, 0, 0, 0, 0, 0, 0, 0, 0, 0, 0, 0, 0, 0, 0, 0, 1] ("Data In")
        # "Universal Reader"
        n69 = call "Initialize.vi"("error in (no error)"=w216, "Node name"="my_node") -> ("error out"=w214:errorcluster)  [unwired: 9 in]
        n70 = call "Create CIF Publisher.vi"("error in (no error)"=w214, "CIF Pcap Publisher Configuration"=T4 {"Name"="Name", "Topic"="Topic", "Link Type"=12356, "Descriptor"="Descipt", "Max Bytes"=100, "Best Effort Subscribers"=1, "Backpressure Subscribers"=0, "Best Effort Queue Depth"=1, "Backpressure Queue Depth"=0}) -> ("error out"=w213:errorcluster, "CIF Publisher Refnum"=w207:T9)  [unwired: 8 in]
        n71 = call "Create CIF Subscriber.vi"("error in (no error)"=w213, "Universal"=TRUE, "CIF Pcap Subscriber Configuration"=T3 {"Name"="Name", "Topic"="Topic", "Link Type"=12345, "Backpressure"=FALSE}) -> ("error out"=w212:errorcluster, "CIF Subscriber Refnum"=w209:T10)  [unwired: 7 in]
        n72 = call "CIF Publish.vi"("CIF Channel Header Publisher"=T2 {"T0"=1, "T_Out"=2, "T_Tx"=3, "ClockID"=4}, "error in (no error)"=w212, "Timeout ms"=u32 1000 ("Timoeut ms"), "Data In"=w195, "Publisher Reference"=w207) -> ("error out"=w211:errorcluster, "Timeout"=w202:bool)  [unwired: 3 in, 2 out]
        n73 = call "CIF Receive.vi"("error in (no error)"=w211, "Timoeut ms"=u32 1000, "Data In"=u8[] [0, 0, 0, 0, 0, 0, 0, 0, 0, 0, 0, 0, 0, 0, 0, 0, 0, 0, 0, 0, 0, 0, 0, 0, 0, 0, 0, 0, 0, 0, 0, 0, 0, 0, 0, 0, 0, 0, 0, 0, 0, 0, 0, 0, 0, 0, 0, 0, 0, 0, 0, 0, 0, 0, 0, 0, 0, 0, 0, 0, 0, 0, 0, 0, 0, 0, 0, 0, 0, 0, 0, 0, 0, 0, 0, 0, 0, 0, 0, 0, 0, 0, 0, 0, 0, 0, 0, 0, 0, 0, 0, 0, 0, 0, 0, 0, 0, 0, 0, 0], "Subscriber Reference"=w209) -> ("error out"=w210:errorcluster, "Array Length"=w194:u32, "Data Out"=w196:u8[], "CIF Channel Header"=w191:T1, "Timeout"=w201:bool)  [unwired: 2 in, 1 out]
        n74 = Equal?(x=w196, y=w195) -> (x = y?=w203:bool)
        n75 = Equal?(x=w194, y=u32 100) -> (x = y?=w192:bool)
        n76 = Equal?(x=w191, y=T1 {"Length"=148, "T0"=1, "T_Out"=2, "T_Tx"=3, "Ctr"=0, "ClockID"=4} ("CIF Channel Header")) -> (x = y?=w190:bool)
        n77 = call "Destroy CIF Subscriber.vi"("error in (no error)"=w210, "Subscriber Reference"=w209) -> ("error out"=w208:errorcluster)  [unwired: 9 in]
        n78 = call "Destroy CIF Publisher.vi"("error in (no error)"=w208, "Publisher Reference"=w207) -> ("error out"=w206:errorcluster)  [unwired: 9 in]
        n79 = Compound Arithmetic op=AND(invert w206, invert w201, invert w202, w203, w192, w190) -> (w217:bool)
        n80 = case shown="True" w217 {
          tunnel: w221 -> [w225 w226]
          tunnel: [w222 w226] -> w220
          tunnel: "Failed Universal Reader" -> [w224 _]
          tunnel: "\r" -> [w223 _]
          frame False {
            n81 = Concatenate Strings(w225, w224, w223) -> (w222:string)
          }
          frame True {
          }
        }
      }
      frame 6 {
        w229 = u8[] [0, 0, 0, 0, 0, 0, 0, 0, 0, 0, 0, 0, 0, 0, 0, 0, 0, 0, 0, 0, 0, 0, 0, 0, 0, 0, 0, 0, 0, 0, 0, 0, 0, 0, 0, 0, 0, 0, 0, 0, 0, 0, 0, 0, 0, 0, 0, 0, 0, 0, 0, 0, 0, 0, 0, 0, 0, 0, 0, 0, 0, 0, 0, 0, 0, 0, 0, 0, 0, 0, 0, 0, 0, 0, 0, 0, 0, 0, 0, 0, 0, 0, 0, 0, 0, 0, 0, 0, 0, 0, 0, 0, 0, 0, 0, 0, 0, 0, 0, 1] ("Data In")
        # "Advanced write"
        n82 = call "Initialize.vi"("error in (no error)"=w257, "Node name"="my_node") -> ("error out"=w255:errorcluster)  [unwired: 9 in]
        n83 = call "Create CIF Publisher.vi"("error in (no error)"=w255, "CIF Pcap Publisher Configuration"=T4 {"Name"="Name", "Topic"="Topic", "Link Type"=12345, "Descriptor"="Descipt", "Max Bytes"=100, "Best Effort Subscribers"=1, "Backpressure Subscribers"=0, "Best Effort Queue Depth"=1, "Backpressure Queue Depth"=0}) -> ("error out"=w254:errorcluster, "CIF Publisher Refnum"=w248:T9)  [unwired: 8 in]
        n84 = call "Create CIF Subscriber.vi"("error in (no error)"=w254, "CIF Pcap Subscriber Configuration"=T3 {"Name"="Name", "Topic"="Topic", "Link Type"=12345, "Backpressure"=FALSE}) -> ("error out"=w253:errorcluster, "CIF Subscriber Refnum"=w250:T10)  [unwired: 8 in]
        n85 = call "CIF Publish.vi"("CIF Publish Advanced"=T6 {"Offset"=25, "Length"=75}, "CIF Channel Header Publisher"=T2 {"T0"=1, "T_Out"=2, "T_Tx"=3, "ClockID"=4}, "error in (no error)"=w253, "Timeout ms"=u32 1000 ("Timoeut ms"), "Data In"=w229, "Publisher Reference"=w248) -> ("error out"=w252:errorcluster, "Timeout"=w243:bool)  [unwired: 2 in, 2 out]
        n86 = Rotate 1D Array(1:w229, 2:-25 ("n")) -> (0:w227:u8[])
        n87 = call "CIF Receive.vi"("error in (no error)"=w252, "Timoeut ms"=u32 1000, "Data In"=u8[] [0, 0, 0, 0, 0, 0, 0, 0, 0, 0, 0, 0, 0, 0, 0, 0, 0, 0, 0, 0, 0, 0, 0, 0, 0, 0, 0, 0, 0, 0, 0, 0, 0, 0, 0, 0, 0, 0, 0, 0, 0, 0, 0, 0, 0, 0, 0, 0, 0, 0, 0, 0, 0, 0, 0, 0, 0, 0, 0, 0, 0, 0, 0, 0, 0, 0, 0, 0, 0, 0, 0, 0, 0, 0, 0, 0, 0, 0, 0, 0, 0, 0, 0, 0, 0, 0, 0, 0, 0, 0, 0, 0, 0, 0, 0, 0, 0, 0, 0, 0], "Subscriber Reference"=w250) -> ("error out"=w251:errorcluster, "Array Length"=w236:u32, "Data Out"=w237:u8[], "CIF Channel Header"=w233:T1, "Timeout"=w242:bool)  [unwired: 2 in, 1 out]
        n88 = Equal?(x=w237, y=w227) -> (x = y?=w244:bool)
        n89 = Equal?(x=w236, y=u32 75) -> (x = y?=w234:bool)
        n90 = Equal?(x=w233, y=T1 {"Length"=123, "T0"=1, "T_Out"=2, "T_Tx"=3, "Ctr"=0, "ClockID"=4} ("CIF Channel Header")) -> (x = y?=w232:bool)
        n91 = call "Destroy CIF Subscriber.vi"("error in (no error)"=w251, "Subscriber Reference"=w250) -> ("error out"=w249:errorcluster)  [unwired: 9 in]
        n92 = call "Destroy CIF Publisher.vi"("error in (no error)"=w249, "Publisher Reference"=w248) -> ("error out"=w247:errorcluster)  [unwired: 9 in]
        n93 = Compound Arithmetic op=AND(invert w247, invert w242, invert w243, w244, w234, w232) -> (w258:bool)
        n94 = case shown="True" w258 {
          tunnel: w262 -> [w266 w267]
          tunnel: [w263 w267] -> w261
          tunnel: "Failed advanced write" -> [w265 _]
          tunnel: "\r" -> [w264 _]
          frame False {
            n95 = Concatenate Strings(w266, w265, w264) -> (w263:string)
          }
          frame True {
          }
        }
      }
      frame 7 {
        w273 = T2 {"T0"=1, "T_Out"=2, "T_Tx"=3, "ClockID"=4} ("CIF Channel Header Publisher")
        w274 = u8[] [0, 0, 0, 0, 0, 0, 0, 0, 0, 0, 0, 0, 0, 0, 0, 0, 0, 0, 0, 0, 0, 0, 0, 0, 0, 0, 0, 0, 0, 0, 0, 0, 0, 0, 0, 0, 0, 0, 0, 0, 0, 0, 0, 0, 0, 0, 0, 0, 0, 0, 0, 0, 0, 0, 0, 0, 0, 0, 0, 0, 0, 0, 0, 0, 0, 0, 0, 0, 0, 0, 0, 0, 0, 0, 0, 0, 0, 0, 0, 0, 0, 0, 0, 0, 0, 0, 0, 0, 0, 0, 0, 0, 0, 0, 0, 0, 0, 0, 0, 1] ("Data In")
        # "Publisher Stats"
        n96 = call "Initialize.vi"("error in (no error)"=w291, "Node name"="my_node") -> ("error out"=w289:errorcluster)  [unwired: 9 in]
        n97 = call "Create CIF Publisher.vi"("error in (no error)"=w289, "CIF Pcap Publisher Configuration"=T4 {"Name"="Name", "Topic"="Topic", "Link Type"=12345, "Descriptor"="Descipt", "Max Bytes"=100, "Best Effort Subscribers"=1, "Backpressure Subscribers"=0, "Best Effort Queue Depth"=1, "Backpressure Queue Depth"=0}) -> ("error out"=w288:errorcluster, "CIF Publisher Refnum"=w275:T9)  [unwired: 8 in]
        n98 = call "Create CIF Subscriber.vi"("error in (no error)"=w288, "CIF Pcap Subscriber Configuration"=T3 {"Name"="Name", "Topic"="Topic", "Link Type"=12345, "Backpressure"=FALSE}) -> ("error out"=w287:errorcluster, "CIF Subscriber Refnum"=w286:T10)  [unwired: 8 in]
        n99 = for {
          N: 100 -> [_]
          tunnel: w275 -> [w302]
          tunnel: u32 1000 ("Timoeut ms") -> [w301]
          tunnel: w273 -> [w300]
          tunnel: w274 -> [w299]
          tunnel: [w298] -> w278
          shift-right: [w297] -> w277
          shift-left: w287 -> [w303]
          n100 = call "CIF Publish.vi"("CIF Channel Header Publisher"=w300, "error in (no error)"=w303, "Timeout ms"=w301, "Data In"=w299, "Publisher Reference"=w302) -> ("error out"=w297:errorcluster, "CIF Publisher Stats"=w298:T7)  [unwired: 3 in, 2 out]
        }
        n101 = call "Reset Stats CIF Publisher.vi"("error in (no error)"=w277, "Publisher Reference"=w275) -> ("error out"=w276:errorcluster)  [unwired: 9 in]
        n102 = Equal?(x=w278, y=T7 {"Writes"=100, "TX Timeouts"=0} ("CIF Publisher Stats")) -> (x = y?=w269:bool)
        n103 = call "CIF Publish.vi"("CIF Channel Header Publisher"=w273, "error in (no error)"=w276, "Data In"=w274, "Publisher Reference"=w275) -> ("error out"=w270:errorcluster, "CIF Publisher Stats"=w272:T7)  [unwired: 4 in, 2 out]
        n104 = Equal?(x=w272, y=T7 {"Writes"=1, "TX Timeouts"=0} ("CIF Publisher Stats")) -> (x = y?=w268:bool)
        n105 = call "Destroy CIF Subscriber.vi"("error in (no error)"=w270, "Subscriber Reference"=w286) -> ("error out"=w285:errorcluster)  [unwired: 9 in]
        n106 = call "Destroy CIF Publisher.vi"("error in (no error)"=w285, "Publisher Reference"=w275) -> ("error out"=w284:errorcluster)  [unwired: 9 in]
        n107 = Compound Arithmetic op=AND(invert w284, w269, w268) -> (w292:bool)
        n108 = case shown="True" w292 {
          tunnel: w296 -> [w307 w308]
          tunnel: [w304 w308] -> w295
          tunnel: "Failed publisher stats" -> [w306 _]
          tunnel: "\r" -> [w305 _]
          frame False {
            n109 = Concatenate Strings(w307, w306, w305) -> (w304:string)
          }
          frame True {
          }
        }
      }
      frame 8 {
        w314 = T2 {"T0"=1, "T_Out"=2, "T_Tx"=3, "ClockID"=4} ("CIF Channel Header Publisher")
        w313 = u8[] [0, 0, 0, 0, 0, 0, 0, 0, 0, 0, 0, 0, 0, 0, 0, 0, 0, 0, 0, 0, 0, 0, 0, 0, 0, 0, 0, 0, 0, 0, 0, 0, 0, 0, 0, 0, 0, 0, 0, 0, 0, 0, 0, 0, 0, 0, 0, 0, 0, 0, 0, 0, 0, 0, 0, 0, 0, 0, 0, 0, 0, 0, 0, 0, 0, 0, 0, 0, 0, 0, 0, 0, 0, 0, 0, 0, 0, 0, 0, 0, 0, 0, 0, 0, 0, 0, 0, 0, 0, 0, 0, 0, 0, 0, 0, 0, 0, 0, 0, 1] ("Data In")
        # "Subscriber Stats"
        n110 = call "Initialize.vi"("error in (no error)"=w332, "Node name"="my_node") -> ("error out"=w330:errorcluster)  [unwired: 9 in]
        n111 = call "Create CIF Publisher.vi"("error in (no error)"=w330, "CIF Pcap Publisher Configuration"=T4 {"Name"="Name", "Topic"="Topic", "Link Type"=12345, "Descriptor"="Descipt", "Max Bytes"=100, "Best Effort Subscribers"=1, "Backpressure Subscribers"=0, "Best Effort Queue Depth"=100, "Backpressure Queue Depth"=0}) -> ("error out"=w329:errorcluster, "CIF Publisher Refnum"=w316:T9)  [unwired: 8 in]
        n112 = call "Create CIF Subscriber.vi"("error in (no error)"=w329, "CIF Pcap Subscriber Configuration"=T3 {"Name"="Name", "Topic"="Topic", "Link Type"=12345, "Backpressure"=FALSE}) -> ("error out"=w315:errorcluster, "CIF Subscriber Refnum"=w310:T10)  [unwired: 8 in]
        n113 = call "CIF Publish.vi"("CIF Channel Header Publisher"=w314, "error in (no error)"=w315, "Data In"=w313, "Publisher Reference"=w316) -> ("error out"=w312:errorcluster, "Data Out"=w311:u8[])  [unwired: 4 in, 2 out]
        n114 = call "CIF Receive.vi"("error in (no error)"=w312, "Data In"=w311, "Subscriber Reference"=w310) -> ("error out"=w309:errorcluster)  [unwired: 3 in, 5 out]
        n115 = for {
          N: 101 -> [_]
          tunnel: w316 -> [w348]
          tunnel: u32 1000 ("Timoeut ms") -> [w347]
          tunnel: w314 -> [w346]
          tunnel: w313 -> [w345]
          tunnel: [w344] -> _
          shift-right: [w343] -> w321
          shift-left: w309 -> [w349]
          n116 = call "CIF Publish.vi"("CIF Channel Header Publisher"=w346, "error in (no error)"=w349, "Timeout ms"=w347, "Data In"=w345, "Publisher Reference"=w348) -> ("error out"=w343:errorcluster, "CIF Publisher Stats"=w344:T7)  [unwired: 3 in, 2 out]
        }
        n117 = for {
          N: 101 -> [_]
          tunnel: w313 -> [w341]
          tunnel: w310 -> [w340]
          tunnel: [w339] -> w319
          shift-right: [w338] -> w320
          shift-left: w321 -> [w342]
          n118 = call "CIF Receive.vi"("error in (no error)"=w342, "Data In"=w341, "Subscriber Reference"=w340) -> ("error out"=w338:errorcluster, "CIF Subscriber Stats"=w339:T8)  [unwired: 3 in, 4 out]
        }
        n119 = Equal?(x=w319, y=T8 {"Reads"=101, "RX Timeouts"=1, "Dropped"=1} ("CIF Subscriber Stats")) -> (x = y?=w322:bool)
        n120 = call "Destroy CIF Subscriber.vi"("error in (no error)"=w320, "Subscriber Reference"=w310) -> ("error out"=w328:errorcluster)  [unwired: 9 in]
        n121 = call "Destroy CIF Publisher.vi"("error in (no error)"=w328, "Publisher Reference"=w316) -> ("error out"=w327:errorcluster)  [unwired: 9 in]
        n122 = Compound Arithmetic op=AND(invert w327, w322) -> (w333:bool)
        n123 = case shown="True" w333 {
          tunnel: w337 -> [w353 w354]
          tunnel: [w350 w354] -> w336
          tunnel: "Failed subscriber stats" -> [w352 _]
          tunnel: "\r" -> [w351 _]
          frame False {
            n124 = Concatenate Strings(w353, w352, w351) -> (w350:string)
          }
          frame True {
          }
        }
      }
      frame 9 {
        w365 = T2 {"T0"=1, "T_Out"=2, "T_Tx"=3, "ClockID"=4} ("CIF Channel Header Publisher")
        w360 = u8[] [0, 0, 0, 0, 0, 0, 0, 0, 0, 0, 0, 0, 0, 0, 0, 0, 0, 0, 0, 0, 0, 0, 0, 0, 0, 0, 0, 0, 0, 0, 0, 0, 0, 0, 0, 0, 0, 0, 0, 0, 0, 0, 0, 0, 0, 0, 0, 0, 0, 0, 0, 0, 0, 0, 0, 0, 0, 0, 0, 0, 0, 0, 0, 0, 0, 0, 0, 0, 0, 0, 0, 0, 0, 0, 0, 0, 0, 0, 0, 0, 0, 0, 0, 0, 0, 0, 0, 0, 0, 0, 0, 0, 0, 0, 0, 0, 0, 0, 0, 1] ("Data In")
        # "Flush"
        n125 = call "Initialize.vi"("error in (no error)"=w380, "Node name"="my_node") -> ("error out"=w378:errorcluster)  [unwired: 9 in]
        n126 = call "Create CIF Publisher.vi"("error in (no error)"=w378, "CIF Pcap Publisher Configuration"=T4 {"Name"="Name", "Topic"="Topic", "Link Type"=12345, "Descriptor"="Descipt", "Max Bytes"=100, "Best Effort Subscribers"=1, "Backpressure Subscribers"=0, "Best Effort Queue Depth"=100, "Backpressure Queue Depth"=0}) -> ("error out"=w377:errorcluster, "CIF Publisher Refnum"=w361:T9)  [unwired: 8 in]
        n127 = call "Create CIF Subscriber.vi"("error in (no error)"=w377, "CIF Pcap Subscriber Configuration"=T3 {"Name"="Name", "Topic"="Topic", "Link Type"=12345, "Backpressure"=FALSE}) -> ("error out"=w355:errorcluster, "CIF Subscriber Refnum"=w364:T10)  [unwired: 8 in]
        n128 = for {
          N: 100 -> [_]
          tunnel: w361 -> [w396]
          tunnel: u32 1000 ("Timoeut ms") -> [w395]
          tunnel: w365 -> [w394]
          tunnel: w360 -> [w393]
          tunnel: [w392] -> _
          shift-right: [w391] -> w363
          shift-left: w355 -> [w397]
          n129 = call "CIF Publish.vi"("CIF Channel Header Publisher"=w394, "error in (no error)"=w397, "Timeout ms"=w395, "Data In"=w393, "Publisher Reference"=w396) -> ("error out"=w391:errorcluster, "CIF Publisher Stats"=w392:T7)  [unwired: 3 in, 2 out]
        }
        n130 = call "Flush CIF Subscriber.vi"("error in (no error)"=w363, "Subscriber Reference"=w364) -> ("error out"=w362:errorcluster, "Discarded"=w358:u32)  [unwired: 8 in]
        n131 = call "CIF Publish.vi"("CIF Channel Header Publisher"=w365, "error in (no error)"=w362, "Data In"=w360, "Publisher Reference"=w361) -> ("error out"=w359:errorcluster)  [unwired: 4 in, 3 out]
        n132 = for {
          N: 2 -> [_]
          tunnel: w360 -> [w389]
          tunnel: w364 -> [w388]
          tunnel: [w387] -> w368
          shift-right: [w386] -> w369
          shift-left: w359 -> [w390]
          n133 = call "CIF Receive.vi"("error in (no error)"=w390, "Data In"=w389, "Subscriber Reference"=w388) -> ("error out"=w386:errorcluster, "CIF Subscriber Stats"=w387:T8)  [unwired: 3 in, 4 out]
        }
        n134 = Equal?(x=w358, y=u32 100) -> (x = y?=w356:bool)
        n135 = Equal?(x=w368, y=T8 {"Reads"=1, "RX Timeouts"=1, "Dropped"=0} ("CIF Subscriber Stats")) -> (x = y?=w370:bool)
        n136 = call "Destroy CIF Subscriber.vi"("error in (no error)"=w369, "Subscriber Reference"=w364) -> ("error out"=w376:errorcluster)  [unwired: 9 in]
        n137 = call "Destroy CIF Publisher.vi"("error in (no error)"=w376, "Publisher Reference"=w361) -> ("error out"=w375:errorcluster)  [unwired: 9 in]
        n138 = Compound Arithmetic op=AND(invert w375, w370, w356) -> (w381:bool)
        n139 = case shown="True" w381 {
          tunnel: w385 -> [w401 w402]
          tunnel: [w398 w402] -> w384
          tunnel: "Failed flush" -> [w400 _]
          tunnel: "\r" -> [w399 _]
          frame False {
            n140 = Concatenate Strings(w401, w400, w399) -> (w398:string)
          }
          frame True {
          }
        }
      }
    }
  }
  "error out" <- w1
  "status" <- w3
  n141 = And Array Elements(Boolean array=w7) -> (logical AND=→"pass":bool)
